vi "test Init Close.vi"(11 "Test Case In":refnum<class "Test Cases.lvclass">) -> (0 "error out":errorcluster, 3 "Test Case Out":refnum<class "Test Cases.lvclass">)   [LabVIEW 2020, in "Test Cases.lvclass"]
uses:
  Test Cases.lvclass
  C:/Program Files/National Instruments/LabVIEW 2026/vi.lib/Astemes/LUnit/Test Case.lvclass
  MyTestHeader/MyTestHeader.lvclass
  D:/git/Sourcegrid-LabVIEW/source/Cells/Cell/Cell.lvclass
  source/Grid/SourceGrid.lvclass
  <vilib>/Astemes/LUnit/Test Case.lvclass/Test Case.ctl
  <vilib>/Astemes/LUnit/Test Case.lvclass
  source/System.Drawing.Color.ctl
  source/SourceGrid.lvlib
  D:/git/Sourcegrid-LabVIEW/source/SourceGrid.dll
  source/SourceGrid.dll
panel:
  in  "Grid Container":refnum<k24>(container)
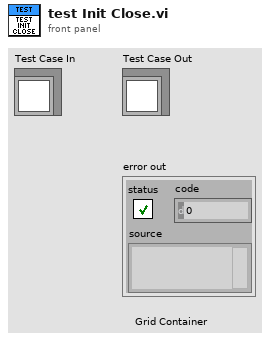
[diagram p1: front panel]
types:
  T1 = typedef "SourceGrid.lvlib/System.Drawing.Color.ctl" = enum16{"AliceBlue", "AntiqueWhite", "Aqua", "Aquamarine", "Azure", "Beige", "Bisque", "Black", "BlanchedAlmond", "Blue", "BlueViolet", "Brown", "BurlyWood", "CadetBlue", "Chartreuse", "Chocolate", "Coral", "CornflowerBlue", "Cornsilk", "Crimson", "Cyan", "DarkBlue", "DarkCyan", "DarkGoldenrod", "DarkGray", "DarkGreen", "DarkKhaki", "DarkMagenta", "DarkOliveGreen", "DarkOrange", "DarkOrchid", "DarkRed", "DarkSalmon", "DarkSeaGreen", "DarkSlateBlue", "DarkSlateGray", "DarkTurquoise", "DarkViolet", "DeepPink", "DeepSkyBlue", "DimGray", "DodgerBlue", "Firebrick", "FloralWhite", "ForestGreen", "Fuchsia", "Gainsboro", "GhostWhite", "Gold", "Goldenrod", "Gray", "Green", "GreenYellow", "Honeydew", "HotPink", "IndianRed", "Indigo", "Ivory", "Khaki", "Lavender", "LavenderBlush", "LawnGreen", "LemonChiffon", "LightBlue", "LightCoral", "LightCyan", "LightGoldenrodYellow", "LightGray", "LightGreen", "LightPink", "LightSalmon", "LightSeaGreen", "LightSkyBlue", "LightSlateGray", "LightSteelBlue", "LightYellow", "Lime", "LimeGreen", "Linen", "Magenta", "Maroon", "MediumAquamarine", "MediumBlue", "MediumOrchid", "MediumPurple", "MediumSeaGreen", "MediumSlateBlue", "MediumSpringGreen", "MediumTurquoise", "MediumVioletRed", "MidnightBlue", "MintCream", "MistyRose", "Moccasin", "NavajoWhite", "Navy", "OldLace", "Olive", "OliveDrab", "Orange", "OrangeRed", "Orchid", "PaleGoldenrod", "PaleGreen", "PaleTurquoise", "PaleVioletRed", "PapayaWhip", "PeachPuff", "Peru", "Pink", "Plum", "PowderBlue", "Purple", "Red", "RosyBrown", "RoyalBlue", "SaddleBrown", "Salmon", "SandyBrown", "SeaGreen", "SeaShell", "Sienna", "Silver", "SkyBlue", "SlateBlue", "SlateGray", "Snow", "SpringGreen", "SteelBlue", "Tan", "Teal", "Thistle", "Tomato", "Transparent", "Turquoise", "Violet", "Wheat", "White", "WhiteSmoke", "Yellow"}
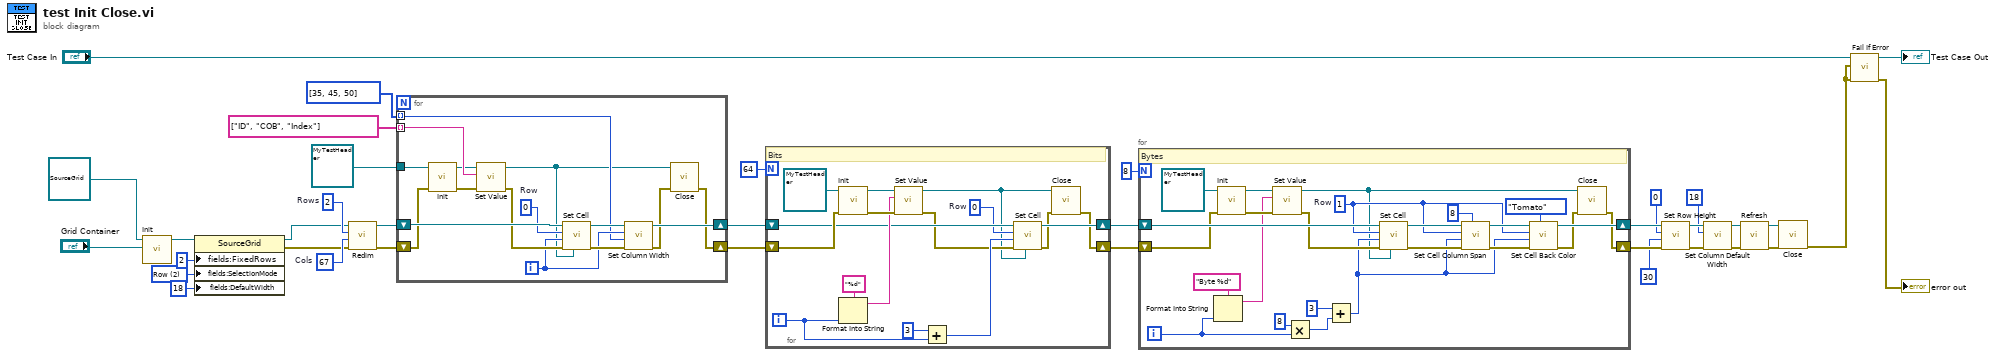
[diagram p0: block diagram]
diagram:
  w30 = 2 items=["Cell"=1, "Row"=2, "Column"=3] ("SelectionMode")
  w31 = 67  # Cols
  w32 = 2  # Rows
  n1 = call-dynamic "Init.vi"("Sourcegrid Container"="Grid Container", "Grid in"=refnum<class "SourceGrid.lvclass"> refnum) -> ("Grid out"=w9:refnum<class "SourceGrid.lvclass">)  [unwired: 8 in, 1 out]
  n2 = property class="SourceGrid"(reference=w9, "fields:FixedRows"=2 ("FixedRows"), "fields:SelectionMode"=w30, "fields:DefaultWidth"=18 ("DefaultWidth")) -> (reference out=w8:refnum<class "SourceGrid.lvclass">, error out=w6:errorcluster)  [unwired: 1 in]
  n3 = call "Redim.vi"("error in"=w6, "Columns"=w31, "Rows"=w32, "Sourcegrid in"=w8) -> ("error out"=w5:errorcluster, "Sourcegrid out"=w7:refnum<class "SourceGrid.lvclass">)  [unwired: 6 in]
  n4 = for {
    shift-right: [w38] -> w22
    shift-left: w5 -> [w49]
    shift-right: [w46] -> w23
    shift-left: w7 -> [w52]
    tunnel: string[] ["ID", "COB", "Index"] -> [w43] mode=indexing
    tunnel: refnum<class "MyTestHeader.lvclass"> refnum ("MyTestHeader.lvclass") -> [w41]
    tunnel: i32[] [35, 45, 50] -> [w44] mode=indexing
    i -> [w45]
    w50 = 0  # Row
    n5 = call-dynamic "Init.vi"("error in"=w49, "MyTestHeader in"=w41) -> ("error out"=w42:errorcluster, "MyTestHeader out"=w40:refnum<class "MyTestHeader.lvclass">)  [unwired: 8 in]
    n6 = call-dynamic "Set Value.vi"("error in"=w42, "Value"=w43, "MyTestHeader in"=w40) -> ("error out"=w48:errorcluster, "MyTestHeader out"=w37:refnum<class "MyTestHeader.lvclass">)  [unwired: 7 in]
    n7 = call "Set Cell.vi"("Cell"=w37, "error in"=w48, "Column"=w45, "Row"=w50, "Sourcegrid in"=w52) -> ("error out"=w51:errorcluster, "Sourcegrid out"=w47:refnum<class "SourceGrid.lvclass">)  [unwired: 5 in]
    n8 = call "Set Column Width.vi"("error in"=w51, "Width"=w44, "Column"=w45, "Sourcegrid in"=w47) -> ("error out"=w39:errorcluster, "Sourcegrid out"=w46:refnum<class "SourceGrid.lvclass">)  [unwired: 6 in]
    n9 = call-dynamic "Close.vi"("error in"=w39, "Cell in"=w37) -> ("error out"=w38:errorcluster)  [unwired: 8 in, 1 out]
  }
  n10 = for {
    N: 64 -> [_]
    shift-right: [w54] -> w19
    shift-left: w22 -> [w66]
    shift-right: [w60] -> w20
    shift-left: w23 -> [w59]
    i -> [w61]
    w58 = 0  # Row
    # "Bits"
    n11 = call-dynamic "Init.vi"("error in"=w66, "MyTestHeader in"=refnum<class "MyTestHeader.lvclass"> refnum ("MyTestHeader.lvclass")) -> ("error out"=w65:errorcluster, "MyTestHeader out"=w64:refnum<class "MyTestHeader.lvclass">)  [unwired: 8 in]
    n12 = Format Into String(format string="%d", w61) -> (resulting string=w63:string)  [unwired: 2 in, 1 out]
    n13 = call-dynamic "Set Value.vi"("error in"=w65, "Value"=w63, "MyTestHeader in"=w64) -> ("error out"=w56:errorcluster, "MyTestHeader out"=w53:refnum<class "MyTestHeader.lvclass">)  [unwired: 7 in]
    n14 = Add(x=3, y=w61) -> (x+y=w57:i32)
    n15 = call "Set Cell.vi"("Cell"=w53, "error in"=w56, "Column"=w57, "Row"=w58, "Sourcegrid in"=w59) -> ("error out"=w55:errorcluster, "Sourcegrid out"=w60:refnum<class "SourceGrid.lvclass">)  [unwired: 5 in]
    n16 = call-dynamic "Close.vi"("error in"=w55, "Cell in"=w53) -> ("error out"=w54:errorcluster)  [unwired: 8 in, 1 out]
  }
  n17 = for {
    N: 8 -> [_]
    shift-right: [w70] -> w18
    shift-left: w19 -> [w87]
    shift-right: [w76] -> w15
    shift-left: w20 -> [w91]
    i -> [w83]
    w74 = 1  # Row
    # "Bytes"
    n18 = Format Into String(format string="Byte %d", w83) -> (resulting string=w81:string)  [unwired: 2 in, 1 out]
    n19 = call-dynamic "Init.vi"("error in"=w87, "MyTestHeader in"=refnum<class "MyTestHeader.lvclass"> refnum ("MyTestHeader.lvclass")) -> ("error out"=w86:errorcluster, "MyTestHeader out"=w89:refnum<class "MyTestHeader.lvclass">)  [unwired: 8 in]
    n20 = call-dynamic "Set Value.vi"("error in"=w86, "Value"=w81, "MyTestHeader in"=w89) -> ("error out"=w85:errorcluster, "MyTestHeader out"=w69:refnum<class "MyTestHeader.lvclass">)  [unwired: 7 in]
    n21 = Multiply(x=8, y=w83) -> (x*y=w80:i32)
    n22 = Add(x=3, y=w80) -> (x+y=w73:i32)
    n23 = call "Set Cell.vi"("Cell"=w69, "error in"=w85, "Column"=w73, "Row"=w74, "Sourcegrid in"=w91) -> ("error out"=w92:errorcluster, "Sourcegrid out"=w79:refnum<class "SourceGrid.lvclass">)  [unwired: 5 in]
    n24 = call "Set Cell Column Span.vi"("Range"=8, "error in"=w92, "Column"=w73, "Row"=w74, "SourceGrid in"=w79) -> ("error out"=w75:errorcluster, "SourceGrid out"=w77:refnum<class "SourceGrid.lvclass">)  [unwired: 5 in]
    n25 = call "Set Cell Back Color.vi"("Color"=System.Drawing.Color."Tomato", "error in"=w75, "Column"=w73, "Row"=w74, "SourceGrid in"=w77) -> ("error out"=w71:errorcluster, "SourceGrid out"=w76:refnum<class "SourceGrid.lvclass">)  [unwired: 5 in]
    n26 = call-dynamic "Close.vi"("error in"=w71, "Cell in"=w69) -> ("error out"=w70:errorcluster)  [unwired: 8 in, 1 out]
  }
  n27 = call "Set Row Height.vi"("error in"=w18, "Height"=30, "Row"=0, "SourceGrid in"=w15) -> ("error out"=w16:errorcluster, "SourceGrid out"=w11:refnum<class "SourceGrid.lvclass">)  [unwired: 6 in]
  n28 = call "Set Column Default Width.vi"("error in"=w16, "Default Width"=18, "SourceGrid in"=w11) -> ("error out"=w24:errorcluster, "SourceGrid out"=w2:refnum<class "SourceGrid.lvclass">)  [unwired: 7 in]
  n29 = call "Refresh.vi"("error in"=w24, "SourceGrid in"=w2) -> ("error out"=w3:errorcluster, "SourceGrid out"=w1:refnum<class "SourceGrid.lvclass">)  [unwired: 8 in]
  n30 = call-dynamic "Close.vi"("error in"=w3, "Sourcegrid in"=w1) -> ("error out"=w27:errorcluster)  [unwired: 8 in, 1 out]
  n31 = call <vilib>:"Fail If Error.vi"("error in (no error)"=w27, "Assert error"=w27, "LUnit Test Case In"="Test Case In") -> ("error out"=→"error out":errorcluster, "LUnit Test Case Out"=→"Test Case Out":refnum<class "Test Cases.lvclass">)  [unwired: 7 in]
